vi "RemoteVI Complex Inspector.vi"() -> ()   [LabVIEW 2020]
doc: "View A of RemoteVI Complex Fixture.vi, shown in its subpanel Viewer. A small panel of its own: Note (string), Count (numeric), Apply (latched button). It obtains the named queue RemoteVI Complex Fixture and enqueues its layout lines (ilayout, RemoteVI Complex Fixture Layout.vi, relative to its panel area) and iorigin x y, where its panel area starts inside its window's client area (Panel Bounds minus RemoteVI Frame Rect.vi of its window); a client finds a control at window x,y + iorigin + ilayout. An event loop enqueues one log line per event: value changes of Note, Count and Apply, key down on Note, mouse down on all three. A parallel loop waits on the named notifier RemoteVI Complex Fixture and, when it fires or is destroyed, sets the hidden switch Inspector Quit with Value (Signaling), which ends the event loop. The fixture writes the queued lines to its log."
uses:
  source/RemoteVI.lvlib
panel:
  in  "Close":bool
  in  "Inspector Quit":bool
  in  "Count":dbl
  in  "Note":string
  in  "Apply":bool
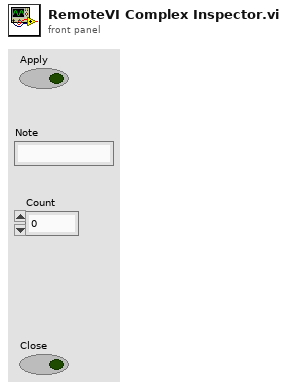
[diagram p1: front panel]
types:
  T1 = typedef "LVRectTypeDef.ctl" = cluster{"left":i16, "top":i16, "right":i16, "bottom":i16}
  T2 = typedef "eventvkey.ctl" = enum16{"ASCII", "Enter", "Return", "Shift", "Ctrl", "Alt", "Cmd", "Opt", "Caps", "NumLock", "Clear", "Break", "Up", "Down", "Left", "Right", "Insert", "Delete", "Home", "End", "PageUp", "PageDown", "Escape", "Help", "Pause", "ScrollLock", "F1", "F2", "F3", "F4", "F5", "F6", "F7", "F8", "F9", "F10", "F11", "F12", "F13", "F14", "F15", "F16", "F17", "F18", "F19", "F20", "F21", "F22", "F23", "F24", "Play", "VolumeUp", "VolumeDown", "Mute", "Two Byte Char"}
  T3 = cluster{"Shift":bool, "Ctrl":bool, "Alt":bool, "Cmd":bool, "Opt":bool}
  T4 = typedef "LVPoint32TypeDef.ctl" = cluster{"Horizontal":i32, "Vertical":i32}
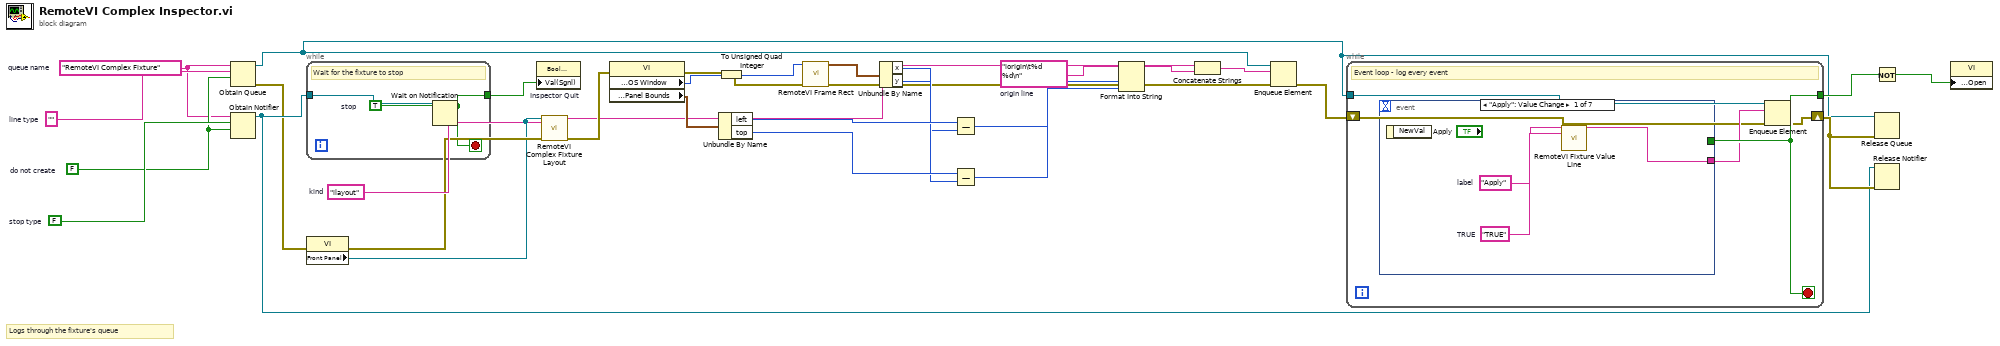
[diagram p0: block diagram]
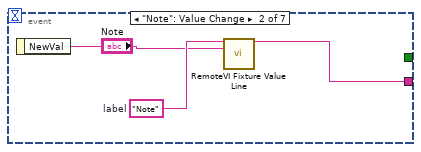
[diagram p2: hidden frame]
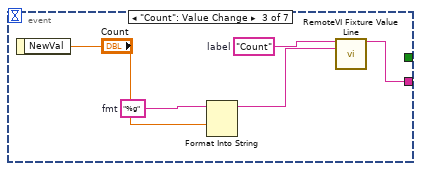
[diagram p3: hidden frame]
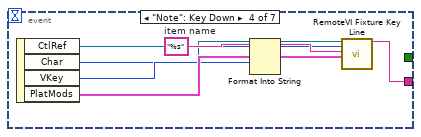
[diagram p4: hidden frame]
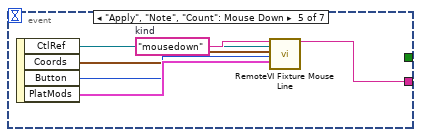
[diagram p5: hidden frame]
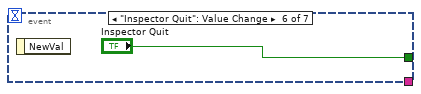
[diagram p6: hidden frame]
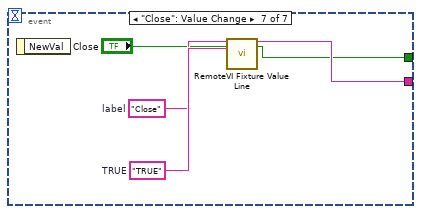
[diagram p7: hidden frame]
diagram:
  w25 = "iorigin\t%d %d\n"  # origin line
  w10 = "ilayout"  # kind
  w6 = FALSE  # stop type
  w3 = FALSE  # do not create
  w2 = ""  # line type
  w1 = "RemoteVI Complex Fixture"  # queue name
  # "Logs through the fixture's queue"
  n1 = Obtain Queue(name (unnamed)=w1, element data type=w2, create if not found? (T)=w3) -> (queue out=w4:refnum<queue>, error out=w5:errorcluster)  [unwired: 2 in, 1 out]
  n2 = Obtain Notifier(name (unnamed)=w1, notification data type=w6, create if not found? (T)=w3) -> (notifier out=w7:refnum<notifier>)  [unwired: 1 in, 2 out]
  n3 = while {
    tunnel: [w34] -> w32
    tunnel: w7 -> [w33]
    stop <- w34 stop-if-true
    w34 = TRUE  # stop
    # "Wait for the fixture to stop"
    n4 = Wait on Notification(notifier=w33) -> ()  [unwired: 3 in, 4 out]
  }
  n5 = property class="VI"(error in=w5) -> (error out=w9:errorcluster, "Front Panel"=w8:refnum<vi>)  [unwired: 1 in, 1 out]
  n6 = property on="Inspector Quit" class="Bool (strict)"("Val(Sgnl)"=w32) -> ()  [unwired: 2 in, 2 out]
  n7 = call "RemoteVI Complex Fixture Layout.vi"("Panel"=w8, "kind"=w10, "Host Panel"=w8, "error in"=w9) -> ("layout"=w11:string, "error out"=w12:errorcluster)  [unwired: 9 in, 1 out]
  n8 = property class="VI"(error in=w12) -> (error out=w15:errorcluster, "Front Panel Window:OS Window"=w13:i32, "Front Panel Window:Panel Bounds"=w14:T1)  [unwired: 1 in, 1 out]
  n9 = To Unsigned Quad Integer(1:w13) -> (0:w16:u64)
  n10 = Unbundle By Name(w14) -> ("left"=w21:i16, "top"=w22:i16)
  n11 = call "RemoteVI Frame Rect.vi"("hWnd"=w16, "error in"=w15) -> ("rect"=w17:cluster{"x":i32, "y":i32, "w":i32, "h":i32}, "error out"=w18:errorcluster)  [unwired: 12 in]
  n12 = Unbundle By Name(w17) -> ("x"=w19:i32, "y"=w20:i32)
  n13 = Subtract(x=w21, y=w19) -> (x-y=w23:i32)
  n14 = Subtract(x=w22, y=w20) -> (x-y=w24:i32)
  n15 = Format Into String(format string=w25, w23, w24) -> (resulting string=w26:string)  [unwired: 2 in, 1 out]
  n16 = Concatenate Strings(w11, w26) -> (w27:string)
  n17 = Enqueue Element(queue=w4, element=w27, error in (no error)=w18) -> (error out=w28:errorcluster)  [unwired: 1 in, 2 out]
  n18 = while {
    tunnel: w4 -> [w35]
    tunnel: [w39] -> w30
    shift-right: [w37] -> w29
    shift-left: w28 -> [w36]
    stop <- w39 stop-if-true
    # "Event loop - log every event"
    n19 = event shown="[0] \"Apply\": Value Change" {
      selector: _ -> [_ _ _ _ _ _ _]
      dyn-events: _ -> [_ _ _ _ _ _ _]
      timeout: _ -> [_ _ _ _ _ _ _]
      tunnel: [_ _ _ _ _ "Inspector Quit" "Close"] -> w39
      tunnel: [w42 w45 w50 w57 w63 _ w68] -> w38
      event "Apply": Value Change {
        w41 = "TRUE"  # TRUE
        w40 = "Apply"  # label
        n20 = event-data() -> ()  [unwired: 1 in, 1 out]
        n21 = call "RemoteVI Fixture Value Line.vi"("label"=w40, "value"=w41) -> ("line"=w42:string)  [unwired: 12 in, 1 out]
      }
      event "Note": Value Change {
        w44 = "Note"  # label
        n22 = event-data() -> ("NewVal"=w43:string)  [unwired: 1 in]
        n23 = call "RemoteVI Fixture Value Line.vi"("label"=w44, "value"=w43) -> ("line"=w45:string)  [unwired: 12 in, 1 out]
      }
      event "Count": Value Change {
        w49 = "Count"  # label
        w47 = "%g"  # fmt
        n24 = event-data() -> ("NewVal"=w46:dbl)  [unwired: 1 in]
        n25 = Format Into String(format string=w47, w46) -> (resulting string=w48:string)  [unwired: 2 in, 1 out]
        n26 = call "RemoteVI Fixture Value Line.vi"("label"=w49, "value"=w48) -> ("line"=w50:string)  [unwired: 12 in, 1 out]
      }
      event "Note": Key Down {
        w55 = "%s"  # item name
        n27 = event-data() -> ("CtlRef"=w51:refnum<vi>, "Char"=w52:i16, "VKey"=w53:T2, "PlatMods"=w54:T3)  [unwired: 1 in]
        n28 = Format Into String(format string=w55, w53) -> (resulting string=w56:string)  [unwired: 2 in, 1 out]
        n29 = call "RemoteVI Fixture Key Line.vi"("CtlRef"=w51, "Char"=w52, "VKey"=w56, "PlatMods"=w54) -> ("line"=w57:string)  [unwired: 14 in, 1 out]
      }
      event "Apply", "Note", "Count": Mouse Down {
        w62 = "mousedown"  # kind
        n30 = event-data() -> ("CtlRef"=w58:refnum<vi>, "Coords"=w59:T4, "Button"=w60:u16, "PlatMods"=w61:T3)  [unwired: 1 in]
        n31 = call "RemoteVI Fixture Mouse Line.vi"("kind"=w62, "CtlRef"=w58, "Coords"=w59, "Button"=w60, "PlatMods"=w61) -> ("line"=w63:string)  [unwired: 13 in, 1 out]
      }
      event "Inspector Quit": Value Change {
        n32 = event-data() -> ()  [unwired: 1 in, 1 out]
      }
      event "Close": Value Change {
        w67 = "TRUE"  # TRUE
        w66 = "Close"  # label
        n33 = event-data() -> ()  [unwired: 1 in, 1 out]
        n34 = call "RemoteVI Fixture Value Line.vi"("label"=w66, "value"=w67) -> ("line"=w68:string)  [unwired: 12 in, 1 out]
      }
    }
    n35 = Enqueue Element(queue=w35, element=w38, error in (no error)=w36) -> (error out=w37:errorcluster)  [unwired: 1 in, 2 out]
  }
  n36 = Not(x=w30) -> (.not. x?=w31:bool)
  n37 = Release Queue(queue=w4, error in (no error)=w29) -> ()  [unwired: 1 in, 3 out]
  n38 = Release Notifier(notifier=w7, error in (no error)=w29) -> ()  [unwired: 1 in, 3 out]
  n39 = property class="VI"("Front Panel Window:Open"=w31) -> ()  [unwired: 2 in, 2 out]
